vi "KYFG Close.vi"(8 "error in (no error)":errorcluster, 11 "handle":u32) -> (0 "error out":errorcluster, 3 "function return":u32(ring))   [LabVIEW 2023, in "KYFGLib_lv.lvlib"]
doc: "KYFG_API FGSTATUS KYFG_Close(FGHANDLE handle);"
uses:
  KYFGLib_lv.lvlib
  KYFGLib.dll
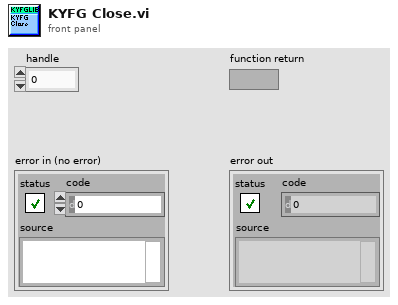
[diagram p1: front panel]
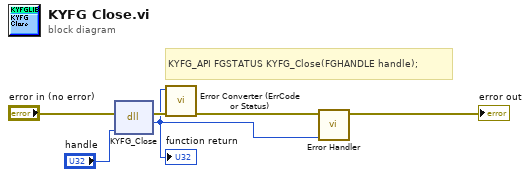
[diagram p0: block diagram]
diagram:
  # "KYFG_API FGSTATUS\tKYFG_Close(FGHANDLE handle);"
  n1 = dll-call lib="KYFGLib.dll" fn="KYFG_Close"(error in="error in (no error)", "handle"="handle") -> (error out=w4:errorcluster, "return type"=w1:u32)  [unwired: 3 in, 1 out]
  "function return" <- w1
  n2 = call "Error Converter (ErrCode or Status).vi"("error in (no error)"=w4, "error code"=w1) -> ("error out"=w3:errorcluster)  [unwired: 9 in]
  n3 = call "Error Handler.vi"("Return Code"=w1, "Error In"=w3) -> ("Error Out"=→"error out":errorcluster)  [unwired: 9 in]
